vi "[ex ce] Differentiation.vi"() -> ()   [LabVIEW 2021]
doc: "CE-Math example.\n\n::: CalcExpress Toolkit :::\nCopyright (c) 2000-2026 Konstantin Shifershteyn. All rights reserved."
uses:
  ce exmpl - 1D difference info.ctl
  <vilib>/gmath/NI_Gmath.lvlib
panel:
  out "max relative difference":T1={"index"=-1, "absolute difference"=0.0, "relative difference, %"=0.0} {"relative difference, %" format="%#.6g"; "absolute difference" format="%#.6g"}
  out "max absolute difference":T1={"index"=-1, "absolute difference"=0.0, "relative difference, %"=0.0} {"relative difference, %" format="%#.6g"; "absolute difference" format="%#.6g"}
  in  "formula info":cluster{"formula":string, "x-variable":string}={"formula"="5*sin(2*x)*exp(-x/3)+2", "x-variable"="x"}
  in  "end":dbl=5.0 format="%.2f"
  in  "start":dbl=-5.0 format="%.2f"
  out "speed ratio":dbl format="%.3f"
  out "GM ticks":u32 caption="ms"
  out "CE ticks":u32 caption="ms"
  out "CE Graph":cluster{"x":dbl[], "f(x)":dbl[]}[](graph) caption="CalcExpress"
  in  "# points":u32=1000
  out "GM Graph":cluster{"x":dbl[], "f(x)":dbl[]}[](graph) caption="G Math"
  # "NOTE    CalcExpress uses (^) operator to perform bitwise-XOR operation but not exponentiation operation.\nYou have to use double-asterisk (**) operator to compute an exponent in a CalcExpress expression. For sample, x**y ."
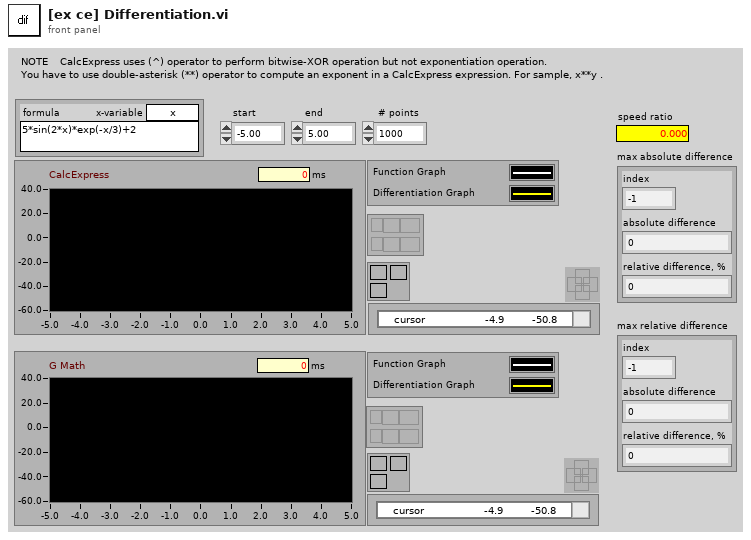
[diagram p1: front panel]
types:
  T1 = typedef "ce exmpl - 1D difference info.ctl" = cluster{"index":i32, "absolute difference":dbl, "relative difference, %":dbl}
  T2 = cluster{"X Values":dbl[], "Derivative of Y":dbl[]}
  T3 = cluster{"X Values":dbl[], "Derivative of Y":dbl[]}[]
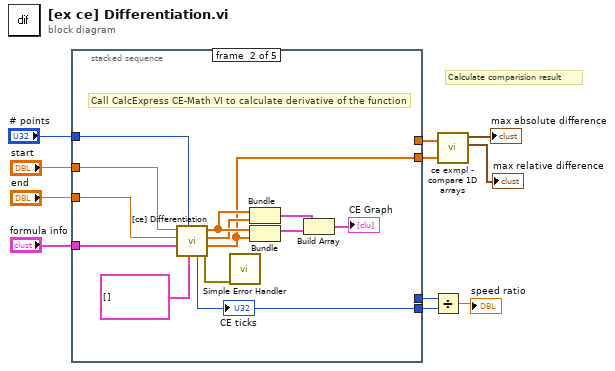
[diagram p0: block diagram]
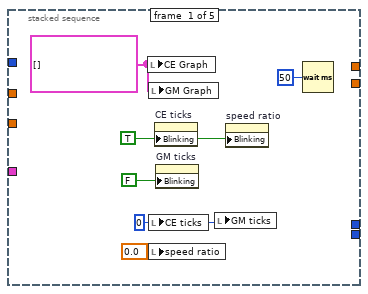
[diagram p2: hidden frame]
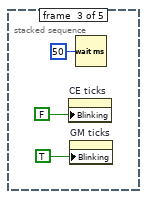
[diagram p3: hidden frame]
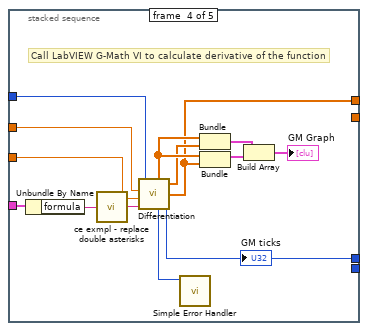
[diagram p4: hidden frame]
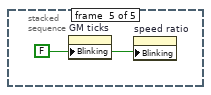
[diagram p5: hidden frame]
diagram:
  # "Calculate comparision result"
  n1 = stacked-sequence {
    tunnel: "start" -> [_ w28 _ w44 _]
    tunnel: "end" -> [_ w27 _ w45 _]
    tunnel: "formula info" -> [_ w26 _ w43 _]
    tunnel: "# points" -> [_ w18 _ w37 _]
    tunnel: [_ w29 _ _ _] -> w11
    tunnel: [_ _ _ w46 _] -> w9
    tunnel: [_ _ _ w36 _] -> w4
    tunnel: [_ w20 _ _ _] -> w3
    frame #0 {
      w12 = cluster{"x":dbl[], "f(x)":dbl[]}[] [] ("CE Graph")
      w14 = u32 0 ("CE ticks")
      w16 = TRUE ("Write Attribute")
      n2 = local write "CE Graph"(w12) -> ()
      n3 = local write "GM Graph"(w12) -> ()
      n4 = local write "CE ticks"(w14) -> ()
      n5 = local write "speed ratio"(0.0 ("speed ratio")) -> ()
      n6 = property on="CE ticks" class="DigNum (strict)"("Blinking"=w16) -> ()  [unwired: 2 in, 2 out]
      n7 = property on="GM ticks" class="DigNum (strict)"("Blinking"=FALSE ("Write Attribute")) -> ()  [unwired: 2 in, 2 out]
      n8 = local write "GM ticks"(w14) -> ()
      n9 = property on="speed ratio" class="DigNum (strict)"("Blinking"=w16) -> ()  [unwired: 2 in, 2 out]
      n10 = Wait (ms)(milliseconds to wait=u32 50) -> ()  [unwired: 1 out]
    }
    frame #1 {
      # "Call CalcExpress CE-Math VI to calculate derivative of the function"
      n11 = call "[ce] Differentiation.vi"("parameters"=cluster{"name":string, "value":dbl}[] [] ("additional parameters"), "# points"=w18, "formula info"=w26, "end"=w27, "start"=w28) -> ("error out"=w30:errorcluster, "Derivative of Y"=w20:dbl[], "Y Values"=w22:dbl[], "X Values"=w23:dbl[], "ticks"=w29:u32)  [unwired: 2 in]
      "CE ticks" <- w29
      n12 = call <vilib>:"Simple Error Handler.vi"("error in (no error)"=w30) -> ()  [unwired: 4 in, 5 out]
      n13 = Bundle("X Values"=w23, "Y Values"=w22) -> (w25:cluster{"X Values":dbl[], "Y Values":dbl[]})  [unwired: 1 in]
      n14 = Bundle("X Values"=w23, "Derivative of Y"=w20) -> (w24:T2)  [unwired: 1 in]
      n15 = Build Array(w25, w24) -> (→"CE Graph":T3)
    }
    frame #2 {
      n16 = property on="CE ticks" class="DigNum (strict)"("Blinking"=FALSE ("Write Attribute")) -> ()  [unwired: 2 in, 2 out]
      n17 = property on="GM ticks" class="DigNum (strict)"("Blinking"=TRUE ("Write Attribute")) -> ()  [unwired: 2 in, 2 out]
      n18 = Wait (ms)(milliseconds to wait=u32 50) -> ()  [unwired: 1 out]
    }
    frame #3 {
      # "Call LabVIEW G-Math VI to calculate derivative of the function"
      n19 = Unbundle By Name(w43) -> ("formula"=w35:string)
      n20 = call "ce exmpl - replace double asterisks .vi"("formula in"=w35) -> ("formula out"=w34:string)  [unwired: 4 in]
      n21 = call <vilib>:"Differentiation.vi"("formula"=w34, "end"=w45, "start"=w44, "number of points"=w37) -> ("ticks"=w46:u32, "error"=w47:i32, "Derivative of Y"=w36:dbl[], "Y Values"=w40:dbl[], "X Values"=w41:dbl[])
      "GM ticks" <- w46
      n22 = call <vilib>:"Simple Error Handler.vi"("error code (no error:0)"=w47) -> ()  [unwired: 4 in, 5 out]
      n23 = Bundle("X Values"=w41, "Y Values"=w40) -> (w39:cluster{"X Values":dbl[], "Y Values":dbl[]})  [unwired: 1 in]
      n24 = Bundle("X Values"=w41, "Derivative of Y"=w36) -> (w38:T2)  [unwired: 1 in]
      n25 = Build Array(w39, w38) -> (→"GM Graph":T3)
    }
    frame #4 {
      w48 = FALSE ("Write Attribute")
      n26 = property on="GM ticks" class="DigNum (strict)"("Blinking"=w48) -> ()  [unwired: 2 in, 2 out]
      n27 = property on="speed ratio" class="DigNum (strict)"("Blinking"=w48) -> ()  [unwired: 2 in, 2 out]
    }
  }
  n28 = Divide(x=w9, y=w11) -> (x/y=→"speed ratio":dbl)
  n29 = call "ce exmpl - compare 1D arrays.vi"("checking array B"=w3, "standard array A"=w4) -> ("max relative difference"=→"max relative difference":T1, "max absolute difference"=→"max absolute difference":T1)  [unwired: 1 in, 2 out]
